vi "RemoteVI VI Of Window.vi"(0 "window":u64) -> (4 "VI":refnum<vi>, 6 "found?":bool)   [LabVIEW 2020, in "RemoteVI.lvlib"]
doc: "The RUNNING VI of this application instance whose front panel window is window (Application:All VIs In Memory, Front Panel Window:OS Window): RemoteVI Server shares a panel of its own LabVIEW as a VI target (tip strips, splitter dragging) and any other window - also the panel of a VI that is not running, which a VI target would stop sharing at once - as a window target. found? is FALSE when no running VI's open panel has that handle; VI is then not a valid refnum. The references of the other VIs are closed; VI stays open (the share uses it). Errors of single VIs are skipped."
uses:
  RemoteVI.lvlib
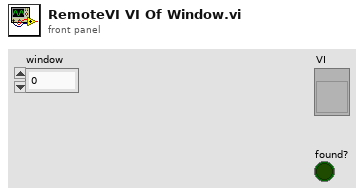
[diagram p1: front panel]
types:
  T1 = enum32{"Bad", "Idle", "Run top level", "Running"}
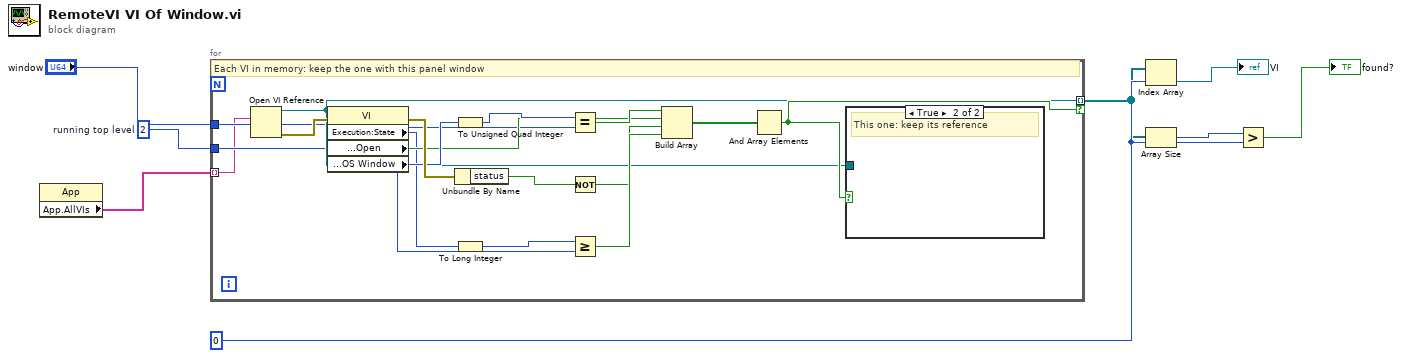
[diagram p0: block diagram]
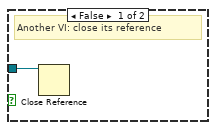
[diagram p2: hidden frame]
diagram:
  w5 = 0
  w3 = 2  # running top level
  n1 = property class="App"() -> ("App.AllVIs"=w2:string[])  [unwired: 2 in, 2 out]
  n2 = for {
    tunnel: "window" -> [w10]
    tunnel: w3 -> [w11]
    tunnel: w2 -> [w9] mode=indexing
    tunnel: [w12] -> w4 mode=indexing if=w25
    # "Each VI in memory: keep the one with this panel window"
    n3 = Open VI Reference(vi path=w9) -> (vi reference=w12:refnum<vi>, error out=w13:errorcluster)  [unwired: 5 in]
    n4 = property class="VI"(reference=w12, error in=w13) -> (error out=w17:errorcluster, "Execution:State"=w14:T1, "Front Panel Window:Open"=w15:bool, "Front Panel Window:OS Window"=w16:i32)  [unwired: 1 out]
    n5 = To Unsigned Quad Integer(1:w16) -> (0:w18:u64)
    n6 = Unbundle By Name(w17) -> ("status"=w20:bool)
    n7 = To Long Integer(number=w14) -> (32bit integer=w22:i32)
    n8 = Equal?(x=w18, y=w10) -> (x = y?=w19:bool)
    n9 = Not(x=w20) -> (.not. x?=w21:bool)
    n10 = Greater Or Equal?(x=w22, y=w11) -> (x >= y?=w23:bool)
    n11 = Build Array(w19, w15, w21, w23) -> (w24:bool[])
    n12 = And Array Elements(Boolean array=w24) -> (logical AND=w25:bool)
    n13 = case shown="True" w25 {
      tunnel: w12 -> [w26 _]
      frame False {
        # "Another VI: close its reference"
        n14 = Close Reference(reference=w26) -> ()  [unwired: 1 in, 1 out]
      }
      frame True {
        # "This one: keep its reference"
      }
    }
  }
  n15 = Index Array(array=w4, index=w5) -> (element=→"VI":refnum<vi>)
  n16 = Array Size(array=w4) -> (size(s)=w7:i32)
  n17 = Greater?(x=w7, y=w5) -> (0:→"found?":bool)
